vi "classify error.vi"(8 "error to classify":errorcluster, 11 "Modbus Slave runtime in":refnum<class "Modbus Module runtime.lvclass">) -> (0 "classified error":errorcluster, 2 "error classification":T1, 3 "Modbus Slave runtime out":refnum<class "Modbus Module runtime.lvclass">)   [LabVIEW 2015, in "Modbus Module runtime.lvclass"]
doc: "Allows a module to classify an error generated at any point during execution. This <b>error classification</b> can then be used by calling code to determine if execution can continue. In addition, this function can be used to allow a component to clear an error, convert an error to a warning, or attempt to recover from an error. Recovery may be attempted only if <b>attempt recovery?</b> is true.Platypus Framework 1.0.1.65\nNI Systems Engineering - National Instruments"
uses:
  Modbus Module runtime.lvclass
  <vilib>/NI/Tag Bus Module Framework/runtime/error classification.ctl
  <vilib>/NI/Tag Bus Module Framework/runtime/TBM module execution interface.lvclass
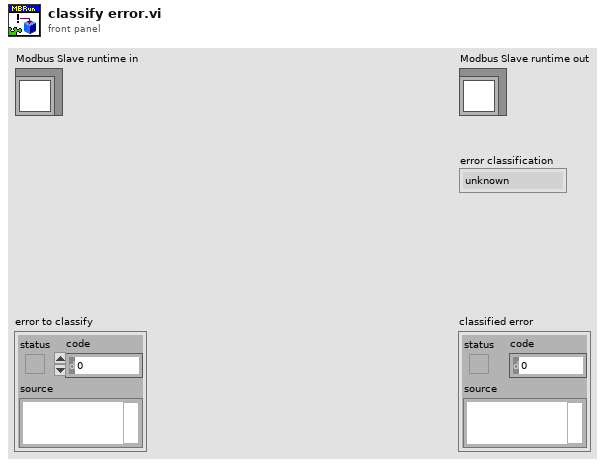
[diagram p1: front panel]
types:
  T1 = typedef "TBM module execution interface.lvclass/error classification.ctl" = enum16{"unknown", "none", "trivial", "recoverable", "critical"}
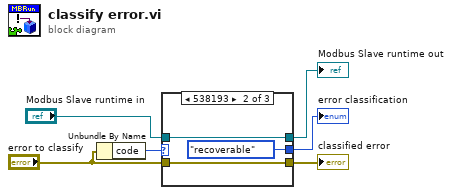
[diagram p0: block diagram]
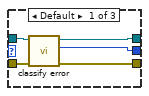
[diagram p2: hidden frame]
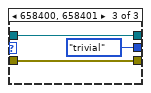
[diagram p3: hidden frame]
diagram:
  n1 = Unbundle By Name("error to classify") -> ("code"=w1:i32)
  n2 = case shown="538193" w1 {
    tunnel: "error to classify" -> [w11 w14 w16]
    tunnel: [w10 w14 w16] -> w6
    tunnel: "Modbus Slave runtime in" -> [w9 w13 w17]
    tunnel: [w8 w13 w17] -> w4
    tunnel: [w7 error_classification."recoverable" ("error classification") error_classification."trivial" ("error classification")] -> w3
    frame Default {
      n3 = call-parent "classify error.vi"("error to classify"=w11, "module in"=w9) -> ("classified error"=w10:errorcluster, "error classification"=w7:T1, "module out"=w8:refnum<class "Modbus Module runtime.lvclass">)  [unwired: 7 in]
    }
    frame 538193 {
    }
    frame 658400, 658401 {
    }
  }
  "Modbus Slave runtime out" <- w4
  "error classification" <- w3
  "classified error" <- w6
